vi "demo.vi"   [LabVIEW 2020]
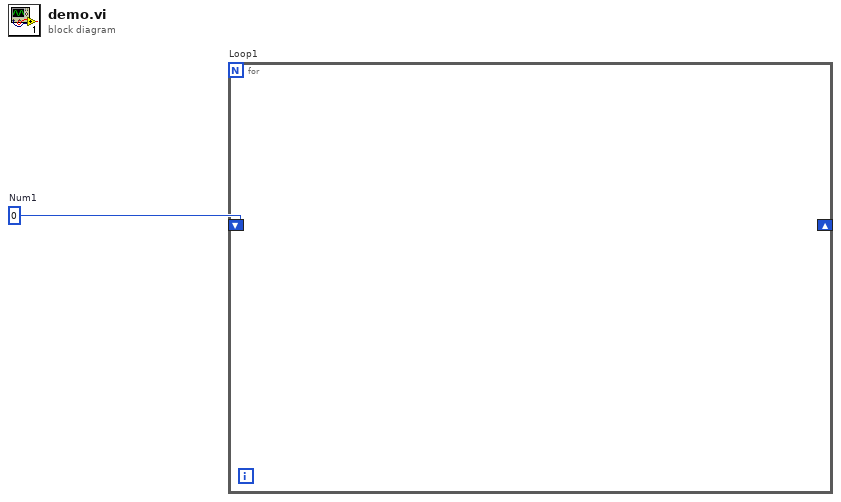
[diagram p0: block diagram]
diagram:
  w1 = 0  # Num1
  n1 = for "Loop1" {
    shift-right: _ -> [_]
    shift-left: w1 -> [_]
  }
